vi "Regex XNode Probe.vi"(0 "input string":string, 5 "regular expression":string, 11 "error in":errorcluster) -> (4 "whole match":string, 6 "matched substrings":string[](array[string]), 15 "error out":errorcluster)   [LabVIEW 2026]
doc: "Probe: Match Regular Expression through the XNode's Execute VI as a plain subVI call."
uses:
  <vilib>/regexp/Match Regular Expression.xnode
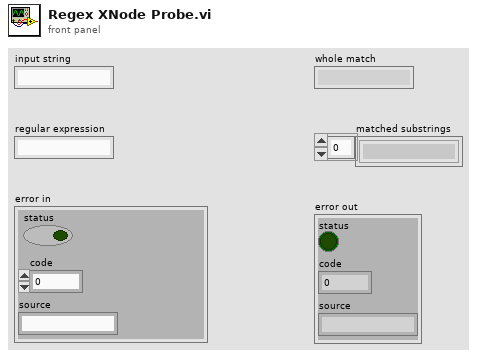
[diagram p1: front panel]
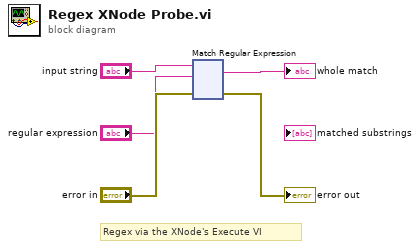
[diagram p0: block diagram]
diagram:
  # "Regex via the XNode's Execute VI"
  n1 = xnode "Match Regular Expression"("input string"="input string", "regular expression"="regular expression", "error in"="error in") -> ("whole match"=→"whole match":string, "error out"=→"error out":errorcluster)  [unwired: 3 in, 3 out]
